vi "Upgrade Addon to Latest Version.vi"(8 "error in (no error)":errorcluster, 11 "Device Item Ref in in":T1 format="%.0x") -> (0 "error out":errorcluster, 3 "Device Item Ref out":T1 format="%.0x")   [LabVIEW 2019, in "FPGA Addon Shared.lvlib"]
uses:
  FPGA Addon Shared.lvlib
  <vilib>/NI VeriStand/Custom Device API/Custom Device Item Ref.ctl
  Types/FG Action.ctl
  Types/Register Information.ctl
  Types/Data Type.ctl
  <vilib>/rvi/FIFO/Fifo_Types/Fifo_DMA_Config.ctl
  <vilib>/rvi/DataTransferAndStorage/Container/Common/niFpgaDataTypeControl.ctl
  <vilib>/rvi/ClientSDK/Core/ModuleGeneration/CommunicationInterfaceUtility/niFpgaDmaChannelImplementation.ctl
  Types/DMA Information.ctl
  NationalInstruments.VeriStand.SystemDefinitionAPI
  Constants.vi
  <vilib>/NI/NI VeriStand Advanced SysDef API/_SubVIs/SysDef.Search.GUID.vi
  <vilib>/NI/NI VeriStand Advanced SysDef API/_SubVIs/SysDef.Property.Get.Variant.vi
  <vilib>/NI/NI VeriStand Advanced SysDef API/SysDef API/SysDef.Property.Set.vi
  <vilib>/NI/NI VeriStand Advanced SysDef API/_SubVIs/SysDef.Property.Set.Variant.vi
  <vilib>/NI/NI VeriStand Advanced SysDef API/_SubVIs/SysDef.Search.GUIDs.vi
  <vilib>/NI/NI VeriStand Advanced SysDef API/SysDef API/Advanced System Definition.lvlib
  <vilib>/NI VeriStand/Custom Device API/Custom Device API.lvlib
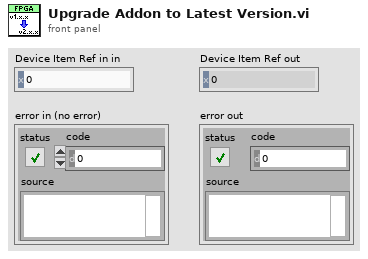
[diagram p1: front panel]
types:
  T1 = typedef "Custom Device API.lvlib/Custom Device Item Ref.ctl" = u64
  T2 = typedef "FPGA Addon Shared.lvlib/FG Action.ctl" = enum8{"GET", "SET"}
  T3 = typedef "FPGA Addon Shared.lvlib/Register Information.ctl" = cluster{"Name":string, "Data Type":T4, "Default Value":variant}
  T4 = typedef "FPGA Addon Shared.lvlib/Data Type.ctl" = enum8{"<Null>", "I8", "I16", "I32", "I64", "U8", "U16", "U32", "U64", "SGL", "Boolean", "Analog PWM In Settings", "Analog PWM In", "Digital PWM In Settings", "Digital PWM In", "Digital PWM Out", "Sine Out", "FXP+/-24.5", "FXP+/-16.5", "FXP+/-32.8", "FXP+/-64.32", "FXP+/-16.7", "FXP+/-20.5", "FXP+/-27.5", "FXP+/-32.16", "FXP+16.3", "FXP+18.3", "Digital Static In", "Digital Static Out", "Digital Static In Settings", "Digital WSS Out", "Quad Encoder Settings", "Quad Encoder In", "Group"}
  T5 = typedef "FPGA Addon Shared.lvlib/DMA Information.ctl" = cluster{"Name":string, "Data Type":T4}
  T6 = cluster{"Name":string, "Data Type":enum8{"<Null>", "I8", "I16", "I32", "I64", "U8", "U16", "U32", "U64", "SGL", "DBL", "EXT", "CSG", "CDB", "CXT", "0x0F", "0x10", "0x11", "0x12", "0x13", "0x14", "Enum U8", "Enum U16", "Enum U32", "Enum U64", "SGL PQ", "DBL PQ", "EXT PQ", "CSG PQ", "CDB PQ", "CXT PQ", "0x1F", "0x20", "Boolean", "0x22", "0x23", "0x24", "0x25", "0x26", "0x27", "0x28", "0x29", "0x2A", "0x2B", "0x2C", "0x2D", "0x2E", "0x2F", "String", "0x31", "Path", "Pict", "0x34", "0x35", "0x36", "DAQ", "0x38", "0x39", "0x3A", "0x3B", "0x3C", "0x3D", "0x3E", "0x3F", "Array", "0x41", "0x42", "0x43", "0x44", "0x45", "0x46", "0x47", "0x48", "0x49", "0x4A", "0x4B", "0x4C", "0x4D", "0x4E", "0x4F", "Cluster", "0x51", "0x52", "Variant", "Waveform", "0x55", "0x56", "0x57", "0x58", "0x59", "0x5A", "0x5B", "0x5C", "0x5D", "0x5E", "0x5F", "0x60", "0x61", "0x62", "0x63", "0x64", "0x65", "0x66", "0x67", "0x68", "0x69", "0x6A", "0x6B", "0x6C", "0x6D", "0x6E", "0x6F", "Refnum"}, "Default Value":dbl}[]
  T7 = enum8{"<Null>", "I8", "I16", "I32", "I64", "U8", "U16", "U32", "U64", "SGL", "DBL", "EXT", "CSG", "CDB", "CXT", "0x0F", "0x10", "0x11", "0x12", "0x13", "0x14", "Enum U8", "Enum U16", "Enum U32", "Enum U64", "SGL PQ", "DBL PQ", "EXT PQ", "CSG PQ", "CDB PQ", "CXT PQ", "0x1F", "0x20", "Boolean", "0x22", "0x23", "0x24", "0x25", "0x26", "0x27", "0x28", "0x29", "0x2A", "0x2B", "0x2C", "0x2D", "0x2E", "0x2F", "String", "0x31", "Path", "Pict", "0x34", "0x35", "0x36", "DAQ", "0x38", "0x39", "0x3A", "0x3B", "0x3C", "0x3D", "0x3E", "0x3F", "Array", "0x41", "0x42", "0x43", "0x44", "0x45", "0x46", "0x47", "0x48", "0x49", "0x4A", "0x4B", "0x4C", "0x4D", "0x4E", "0x4F", "Cluster", "0x51", "0x52", "Variant", "Waveform", "0x55", "0x56", "0x57", "0x58", "0x59", "0x5A", "0x5B", "0x5C", "0x5D", "0x5E", "0x5F", "0x60", "0x61", "0x62", "0x63", "0x64", "0x65", "0x66", "0x67", "0x68", "0x69", "0x6A", "0x6B", "0x6C", "0x6D", "0x6E", "0x6F", "Refnum"}
  T8 = typedef "Fifo_DMA_Config.ctl" = cluster{"Name":string, "Depth":u32, "Write? (Deprecated:Use Implementation)":bool, "Physical Channel":u32, "Base Address":u32, "Data Width":u32, "Data Type":T9, "FXP Properties":variant, "Write Window Address":u32, "Implementation":T10, "Control Set":u32}
  T9 = typedef "niFpgaDataTypeControl.ctl" = enum32{"Boolean", "I8", "I16", "I32", "I64", "U8", "U16", "U32", "U64", "FXP", "CustomControl", "SGL"}
  T10 = typedef "niFpgaDmaChannelImplementation.ctl" = enum16{"niFpgaTargetToHost", "niFpgaHostToTarget", "niFpgaPeerToPeerWriter", "niFpgaPeerToPeerReader", "niCoreTargetToHost", "niCoreHostToTarget"}
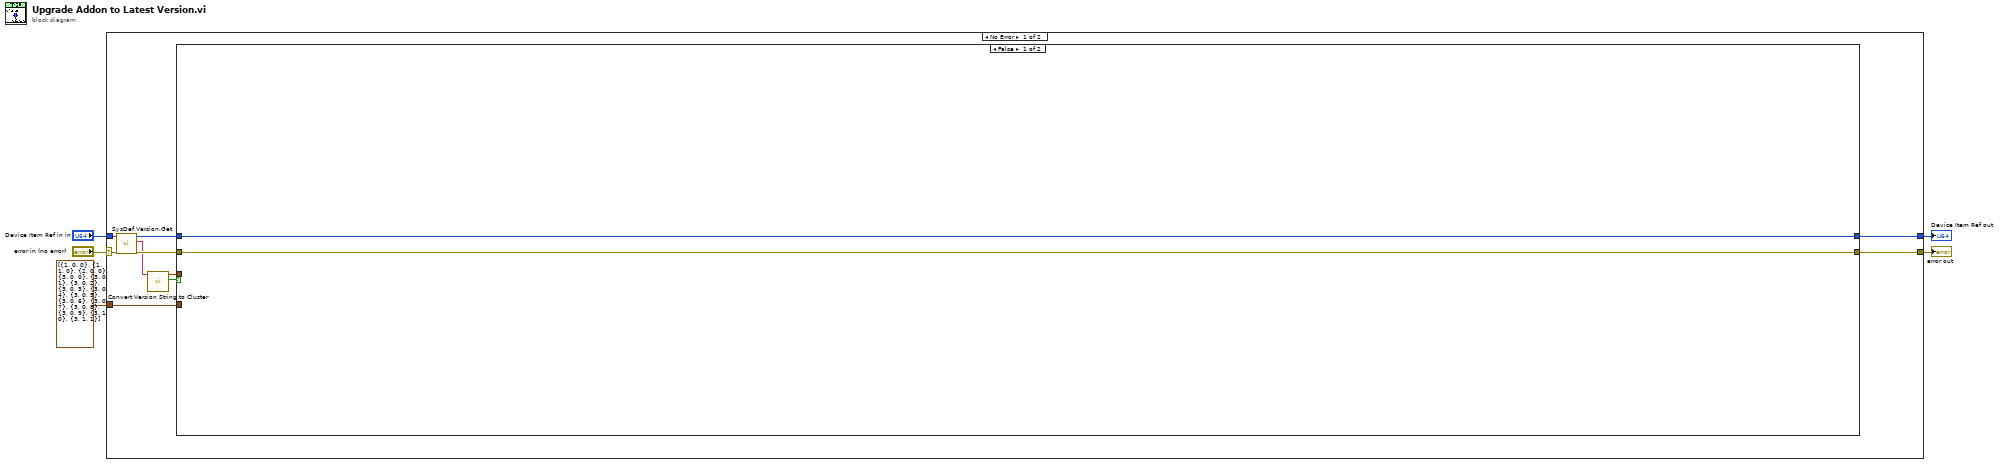
[diagram p0: block diagram]
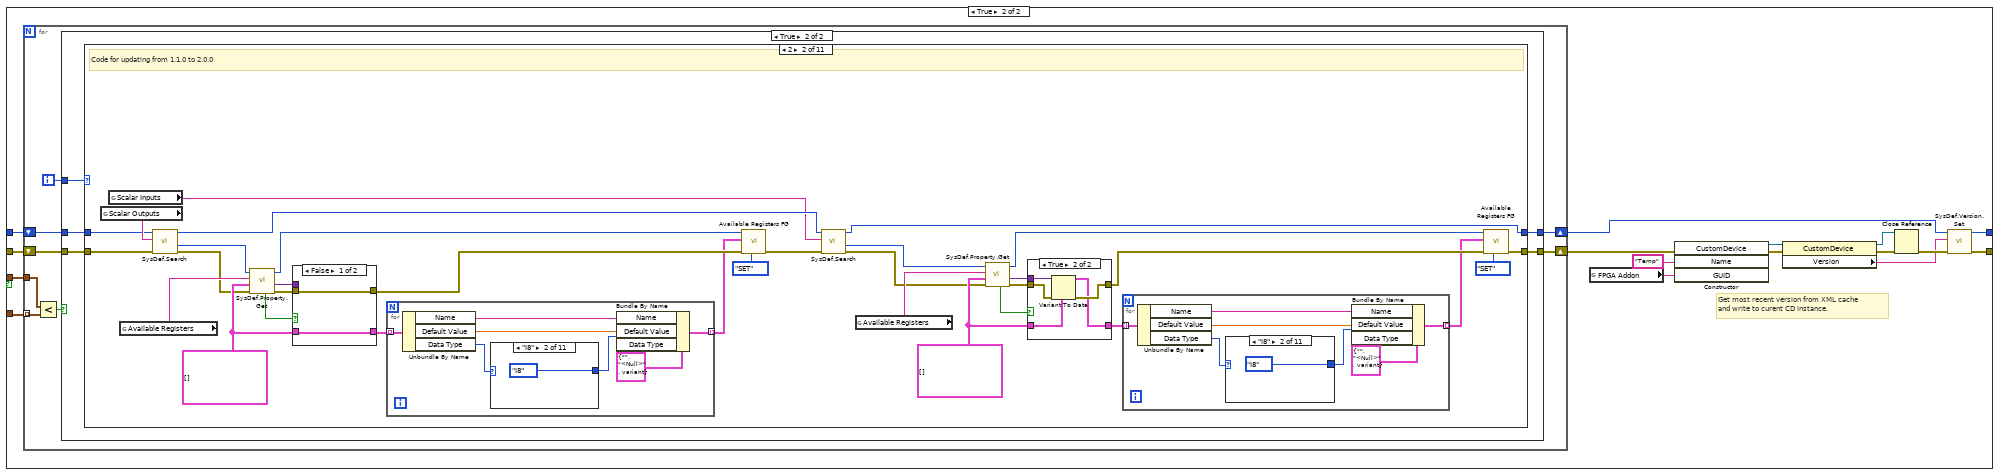
[diagram p2: hidden frame]
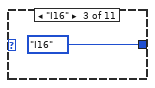
[diagram p6: hidden frame]
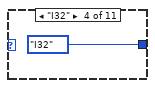
[diagram p7: hidden frame]
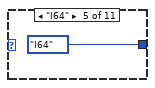
[diagram p8: hidden frame]
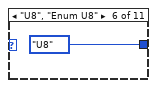
[diagram p9: hidden frame]
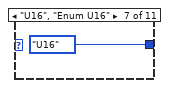
[diagram p10: hidden frame]
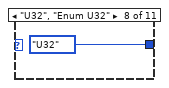
[diagram p11: hidden frame]
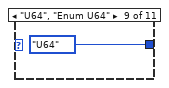
[diagram p12: hidden frame]
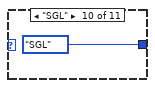
[diagram p13: hidden frame]
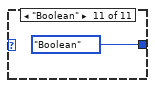
[diagram p14: hidden frame]
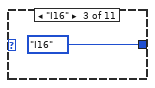
[diagram p17: hidden frame]
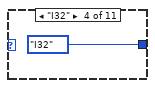
[diagram p18: hidden frame]
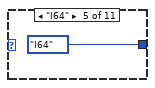
[diagram p19: hidden frame]
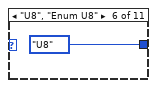
[diagram p20: hidden frame]
diagram:
  n1 = case shown="No Error" "error in (no error)" {
    selector: "error in (no error)" -> [w13 w213]
    tunnel: [w15 w213] -> w4
    tunnel: "Device Item Ref in in" -> [w12 w212]
    tunnel: [w14 w212] -> w5
    tunnel: cluster{i32, i32, i32}[] [{1, 0, 0}, {1, 1, 0}, {2, 0, 0}, {3, 0, 0}, {3, 0, 1}, {3, 0, 2}, {3, 0, 3}, {3, 0, 4}, {3, 0, 5}, {3, 0, 6}, {3, 0, 7}, {3, 0, 8}, {3, 0, 9}, {3, 1, 0}, {3, 1, 1}] -> [w9 _]
    frame No Error {
      n2 = call <vilib>:"SysDef.Version.Get.vi"("error in (no error)"=w13, "nodeID"=w12) -> ("error out"=w10:errorcluster, "Version"=w8:string, "nodeID out"=w11:u64)  [unwired: 7 in]
      n3 = call "Convert Version String to Cluster.vi"("Version"=w8) -> ("Version Valid?"=w6:bool, "Version"=w7:cluster{i32, i32, i32})  [unwired: 9 in]
      n4 = case shown="False" w6 {
        tunnel: [w17 w27] -> w15
        tunnel: [w16 w26] -> w14
        tunnel: w11 -> [w16 w21]
        tunnel: w10 -> [w17 w20]
        tunnel: w9 -> [_ w19]
        tunnel: w7 -> [_ w18]
        frame False {
        }
        frame True {
          # "Get most recent version from XML cache\nand write to curent CD instance."
          n5 = for {
            shift-right: [w41] -> w24
            shift-left: w20 -> [w34]
            shift-right: [w40] -> w25
            shift-left: w21 -> [w35]
            tunnel: w18 -> [w38]
            tunnel: w19 -> [w36] mode=indexing
            i -> [w39]
            n6 = Less?(x=w38, y=w36) -> (x < y?=w37:bool)
            n7 = case shown="True" w37 {
              tunnel: w34 -> [w43 w48]
              tunnel: [w43 w47] -> w41
              tunnel: w35 -> [w42 w44]
              tunnel: [w42 w45] -> w40
              tunnel: w39 -> [_ w46]
              frame False {
              }
              frame True {
                n8 = case shown="2" w46 {
                  tunnel: w48 -> [w50 w76 w156 w188 w190 w192 w194 w196 w203 w209 w211]
                  tunnel: [w50 w51 w132 w188 w190 w192 w194 w196 w198 w209 w211] -> w47
                  tunnel: [w49 w52 w133 w187 w189 w191 w193 w195 w197 w208 w210] -> w45
                  tunnel: w44 -> [w49 w75 w155 w187 w189 w191 w193 w195 w202 w208 w210]
                  frame Default {
                  }
                  frame 2 {
                    w59 = T6 [] ("Available Registers 2")
                    w70 = T6 [] ("Available Registers 2")
                    # "Code for updating from 1.1.0 to 2.0.0"
                    n9 = global read "Constants.vi" "Scalar Outputs"() -> (w81:string)
                    n10 = global read "Constants.vi" "Scalar Inputs"() -> (w77:string)
                    n11 = global read "Constants.vi" "Available Registers"() -> (w71:string)
                    n12 = call-poly <vilib>:"SysDef.Search.vi"("error in (no error)"=w76, "GUID"=w81, "nodeID"=w75) -> ("error out"=w67:errorcluster, "Value out"=w69:u64, "nodeID out"=w78:u64)  [unwired: 5 in, 1 out]
                    n13 = call-poly <vilib>:"SysDef.Property.Get.vi"("error in (no error)"=w67, "Value"=w70, "Property Name"=w71, "nodeID"=w69) -> ("error out"=w73:errorcluster, "Value"=w72:variant, "nodeID out"=w68:u64, "Found?"=w74:bool)  [unwired: 4 in]
                    n14 = case shown="False" w74 {
                      tunnel: w72 -> [_ w130]
                      tunnel: w70 -> [w124 w129]
                      tunnel: w73 -> [w125 w128]
                      tunnel: [w125 w127] -> w66
                      tunnel: [w124 w126] -> w65
                      frame False {
                      }
                      frame True {
                        n15 = Variant To Data(error in=w128, type=w129, Variant=w130) -> (data=w126:T6, error out=w127:errorcluster)
                      }
                    }
                    n16 = for {
                      tunnel: w65 -> [w113] mode=indexing
                      tunnel: [w109] -> w64 mode=indexing
                      n17 = Unbundle By Name(w113) -> ("Name"=w112:string, "Default Value"=w111:dbl, "Data Type"=w108:T7)
                      n18 = case shown="\"I8\"" w108 {
                        tunnel: [_ Data_Type."I8" ("Data Type") Data_Type."I16" ("Data Type") Data_Type."I32" ("Data Type") Data_Type."I64" ("Data Type") Data_Type."U8" ("Data Type") Data_Type."U16" ("Data Type") Data_Type."U32" ("Data Type") Data_Type."U64" ("Data Type") Data_Type."SGL" ("Data Type") Data_Type."Boolean" ("Data Type")] -> w107
                        frame Default {
                        }
                        frame "I8" {
                        }
                        frame "I16" {
                        }
                        frame "I32" {
                        }
                        frame "I64" {
                        }
                        frame "U8", "Enum U8" {
                        }
                        frame "U16", "Enum U16" {
                        }
                        frame "U32", "Enum U32" {
                        }
                        frame "U64", "Enum U64" {
                        }
                        frame "SGL" {
                        }
                        frame "Boolean" {
                        }
                      }
                      n19 = Bundle By Name(cluster=T3 {"Name"="", "Data Type"=enum."<Null>", "Default Value"=variant(refnum<class> refnum)}, "Name"=w112, "Default Value"=w111, "Data Type"=w107) -> (w109:T3)
                    }
                    n20 = call "Available Registers FG.vi"("Action"=FG_Action."SET", "error in (no error)"=w66, "Available Registers"=w64, "Item Ref"=w68) -> ("error out"=w79:errorcluster)  [unwired: 5 in, 2 out]
                    n21 = call-poly <vilib>:"SysDef.Search.vi"("error in (no error)"=w79, "GUID"=w77, "nodeID"=w78) -> ("error out"=w57:errorcluster, "Value out"=w54:u64, "nodeID out"=w52:u64)  [unwired: 5 in, 1 out]
                    n22 = global read "Constants.vi" "Available Registers"() -> (w60:string)
                    n23 = call-poly <vilib>:"SysDef.Property.Get.vi"("error in (no error)"=w57, "Value"=w59, "Property Name"=w60, "nodeID"=w54) -> ("error out"=w62:errorcluster, "Value"=w61:variant, "nodeID out"=w53:u64, "Found?"=w63:bool)  [unwired: 4 in]
                    n24 = case shown="True" w63 {
                      tunnel: w61 -> [_ w106]
                      tunnel: w59 -> [w100 w105]
                      tunnel: w62 -> [w101 w104]
                      tunnel: [w101 w103] -> w56
                      tunnel: [w100 w102] -> w58
                      frame False {
                      }
                      frame True {
                        n25 = Variant To Data(error in=w104, type=w105, Variant=w106) -> (data=w102:T6, error out=w103:errorcluster)
                      }
                    }
                    n26 = for {
                      tunnel: w58 -> [w89] mode=indexing
                      tunnel: [w85] -> w55 mode=indexing
                      n27 = Unbundle By Name(w89) -> ("Name"=w88:string, "Default Value"=w87:dbl, "Data Type"=w84:T7)
                      n28 = case shown="\"I8\"" w84 {
                        tunnel: [_ Data_Type."I8" ("Data Type") Data_Type."I16" ("Data Type") Data_Type."I32" ("Data Type") Data_Type."I64" ("Data Type") Data_Type."U8" ("Data Type") Data_Type."U16" ("Data Type") Data_Type."U32" ("Data Type") Data_Type."U64" ("Data Type") Data_Type."SGL" ("Data Type") Data_Type."Boolean" ("Data Type")] -> w83
                        frame Default {
                        }
                        frame "I8" {
                        }
                        frame "I16" {
                        }
                        frame "I32" {
                        }
                        frame "I64" {
                        }
                        frame "U8", "Enum U8" {
                        }
                        frame "U16", "Enum U16" {
                        }
                        frame "U32", "Enum U32" {
                        }
                        frame "U64", "Enum U64" {
                        }
                        frame "SGL" {
                        }
                        frame "Boolean" {
                        }
                      }
                      n29 = Bundle By Name(cluster=T3 {"Name"="", "Data Type"=enum."<Null>", "Default Value"=variant(refnum<class> refnum)}, "Name"=w88, "Default Value"=w87, "Data Type"=w83) -> (w85:T3)
                    }
                    n30 = call "Available Registers FG.vi"("Action"=FG_Action."SET", "error in (no error)"=w56, "Available Registers"=w55, "Item Ref"=w53) -> ("error out"=w51:errorcluster)  [unwired: 5 in, 2 out]
                  }
                  frame 5 {
                    w131 = T8[] [] ("Available Registers 2")
                    w140 = T8[] [] ("Available Registers 2")
                    # "Code for updating from 3.0.1 to 3.0.2"
                    n31 = global read "Constants.vi" "Waveform Outputs"() -> (w157:string)
                    n32 = global read "Constants.vi" "Waveform Inputs"() -> (w161:string)
                    n33 = global read "Constants.vi" "Available DMA"() -> (w151:string)
                    n34 = call-poly <vilib>:"SysDef.Search.vi"("error in (no error)"=w156, "GUID"=w161, "nodeID"=w155) -> ("error out"=w148:errorcluster, "Value out"=w150:u64, "nodeID out"=w158:u64)  [unwired: 5 in, 1 out]
                    n35 = call-poly <vilib>:"SysDef.Property.Get.vi"("error in (no error)"=w148, "Value"=w131, "Property Name"=w151, "nodeID"=w150) -> ("error out"=w153:errorcluster, "Value"=w152:variant, "nodeID out"=w149:u64, "Found?"=w154:bool)  [unwired: 4 in]
                    n36 = case shown="False" w154 {
                      tunnel: w152 -> [_ w186]
                      tunnel: w131 -> [w180 w185]
                      tunnel: w153 -> [w181 w184]
                      tunnel: [w181 w183] -> w147
                      tunnel: [w180 w182] -> w146
                      frame False {
                      }
                      frame True {
                        n37 = Variant To Data(error in=w184, type=w185, Variant=w186) -> (data=w182:T8[], error out=w183:errorcluster)
                      }
                    }
                    n38 = for {
                      tunnel: w146 -> [w179] mode=indexing
                      tunnel: [w177] -> w145 mode=indexing
                      n39 = Unbundle By Name(w179) -> ("Name"=w178:string)
                      n40 = Bundle By Name(cluster=T5 {"Name"="", "Data Type"=enum."<Null>"} ("Cluster"), "Name"=w178, "Data Type"=Data_Type."SGL") -> (w177:T5)
                    }
                    n41 = call "Available DMA FG.vi"("Action"=FG_Action."SET", "error in (no error)"=w147, "Available DMA"=w145, "Item Ref"=w149) -> ("error out"=w159:errorcluster)  [unwired: 5 in, 2 out]
                    n42 = call-poly <vilib>:"SysDef.Search.vi"("error in (no error)"=w159, "GUID"=w157, "nodeID"=w158) -> ("error out"=w138:errorcluster, "Value out"=w135:u64, "nodeID out"=w133:u64)  [unwired: 5 in, 1 out]
                    n43 = global read "Constants.vi" "Available DMA"() -> (w141:string)
                    n44 = call-poly <vilib>:"SysDef.Property.Get.vi"("error in (no error)"=w138, "Value"=w140, "Property Name"=w141, "nodeID"=w135) -> ("error out"=w143:errorcluster, "Value"=w142:variant, "nodeID out"=w134:u64, "Found?"=w144:bool)  [unwired: 4 in]
                    n45 = case shown="False" w144 {
                      tunnel: w142 -> [_ w174]
                      tunnel: w140 -> [w168 w173]
                      tunnel: w143 -> [w169 w172]
                      tunnel: [w169 w171] -> w137
                      tunnel: [w168 w170] -> w139
                      frame False {
                      }
                      frame True {
                        n46 = Variant To Data(error in=w172, type=w173, Variant=w174) -> (data=w170:T8[], error out=w171:errorcluster)
                      }
                    }
                    n47 = for {
                      tunnel: w139 -> [w167] mode=indexing
                      tunnel: [w165] -> w136 mode=indexing
                      n48 = Unbundle By Name(w167) -> ("Name"=w166:string)
                      n49 = Bundle By Name(cluster=T5 {"Name"="", "Data Type"=enum."<Null>"} ("Cluster"), "Name"=w166, "Data Type"=Data_Type."SGL") -> (w165:T5)
                    }
                    n50 = call "Available DMA FG.vi"("Action"=FG_Action."SET", "error in (no error)"=w137, "Available DMA"=w136, "Item Ref"=w134) -> ("error out"=w132:errorcluster)  [unwired: 5 in, 2 out]
                  }
                  frame 6 {
                    # "Code for updating from 3.0.2 to 3.0.3"
                  }
                  frame 7 {
                    # "Code for updating from 3.0.3 to 3.0.4"
                  }
                  frame 8 {
                    # "Code for updating from 3.0.4 to 3.0.5"
                  }
                  frame 9 {
                    # "Code for updating from 3.0.5 to 3.0.6"
                  }
                  frame 10 {
                    # "Code for updating from 3.0.6 to 3.0.7"
                  }
                  frame 11 {
                    # "Code for updating from 3.0.8 to 3.0.9"
                    n51 = global read "Constants.vi" "DMA Error"() -> (w201:string)
                    n52 = call-poly <vilib>:"SysDef.Search.vi"("error in (no error)"=w203, "GUID"=w201, "nodeID"=w202) -> ("error out"=w199:errorcluster, "Values Out"=w200:u64[], "nodeID out"=w197:u64)  [unwired: 5 in, 1 out]
                    n53 = for {
                      tunnel: w200 -> [w206] mode=indexing
                      shift-right: [w204] -> w198
                      shift-left: w199 -> [w207]
                      n54 = call <vilib>:"SysDef.Rename.vi"("error in (no error)"=w207, "Name"="Error Code", "nodeID"=w206) -> ("error out"=w204:errorcluster)  [unwired: 6 in, 2 out]
                    }
                  }
                  frame 12 {
                    # "Code for updating from 3.0.9 to 3.1.0"
                  }
                  frame 13 {
                    # "Code for updating from 3.1.0 to 3.1.1"
                  }
                }
              }
            }
          }
          n55 = global read "Constants.vi" "FPGA Addon"() -> (w22:string)
          n56 = constructor class="CustomDevice"(error in=w24, "Name"="Temp", "GUID"=w22) -> (reference out=w33:refnum<k24>, error out=w32:errorcluster)  [unwired: 2 in, 3 out]
          n57 = property class="CustomDevice"(reference=w33, error in=w32) -> (reference out=w30:refnum<k24>, error out=w31:errorcluster, "Version"=w28:string)
          n58 = Close Reference(reference=w30, error in (no error)=w31) -> (error out=w29:errorcluster)
          n59 = call <vilib>:"SysDef.Version.Set.vi"("error in (no error)"=w29, "Version"=w28, "nodeID"=w25) -> ("error out"=w27:errorcluster, "nodeID out"=w26:u64)  [unwired: 7 in]
        }
      }
    }
    frame Error {
    }
  }
  "Device Item Ref out" <- w5
  "error out" <- w4
